vi "Find Analog Replay.vi"(8 "error in (no error)":errorcluster, 9 "RIO Device Address":string, 10 "Name":string, 11 "APU in":refnum<k24>) -> (0 "error out":errorcluster, 2 "Analog Replay":refnum<k24>, 3 "APU out":refnum<k24>)   [LabVIEW 2020, in "Engine Simulation Toolkit Scripting API.lvlib"]
uses:
  Engine Simulation Toolkit Scripting API.lvlib
  NationalInstruments.VeriStand.SystemDefinitionAPI
  Shared/Constants and GUIDs.vi
  Shared/Engine Simulation Toolkit Shared.lvlib
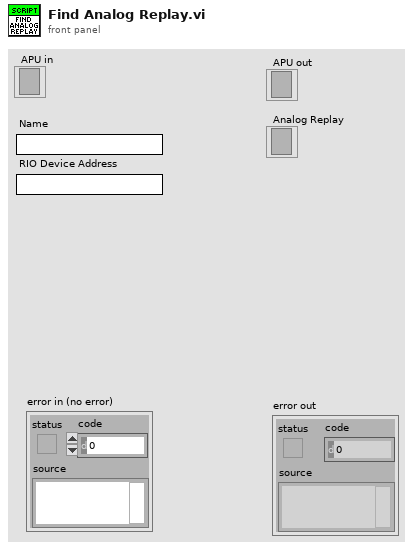
[diagram p1: front panel]
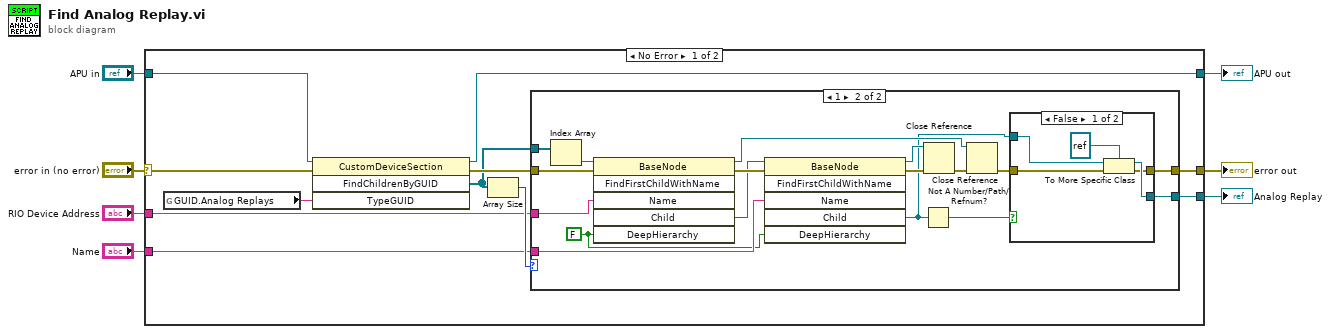
[diagram p0: block diagram]
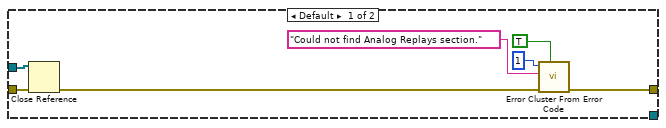
[diagram p2: hidden frame]
diagram:
  n1 = case shown="No Error" "error in (no error)" {
    selector: "error in (no error)" -> [w10 w50]
    tunnel: [w12 w50] -> w7
    tunnel: "APU in" -> [w18 w49]
    tunnel: [w11 w49] -> w4
    tunnel: "RIO Device Address" -> [w13 _]
    tunnel: "Name" -> [w9 _]
    tunnel: [w8 _] -> w1
    frame No Error {
      n2 = global read "Constants and GUIDs.vi" "GUID.Analog Replays"() -> (w17:string)
      n3 = invoke class="CustomDeviceSection" method="FindChildrenByGUID"(reference=w18, error in=w10, "TypeGUID"=w17) -> (reference out=w11:refnum<k24>, error out=w15:errorcluster, "FindChildrenByGUID"=w14:refnum<k24>[])  [unwired: 1 in, 1 out]
      n4 = Array Size(array=w14) -> (size(s)=w16:i32)
      n5 = case shown="1" w16 {
        tunnel: [w25 w27] -> w12
        tunnel: w15 -> [w20 w37]
        tunnel: w14 -> [w21 w42]
        tunnel: w13 -> [_ w40]
        tunnel: w9 -> [_ w32]
        tunnel: [_ w26] -> w8
        frame Default {
          n6 = Close Reference(reference=w21, error in (no error)=w20) -> (error out=w19:errorcluster)
          n7 = call <vilib>:"Error Cluster From Error Code.vi"("show call chain? (False)"=TRUE, "error in (no error)"=w19, "error message (\"\")"="Could not find Analog Replays section." ("error message (\"\")"), "error code (0)"=1) -> ("error out"=w25:errorcluster)  [unwired: 5 in]
        }
        frame 1 {
          w31 = FALSE ("DeepHierarchy")
          n8 = Index Array(array=w42) -> (element=w41:refnum<k24>)  [unwired: 1 in]
          n9 = invoke class="BaseNode" method="FindFirstChildWithName"(reference=w41, error in=w37, "Name"=w40, "DeepHierarchy"=w31) -> (reference out=w33:refnum<k24>, error out=w39:errorcluster, "Child"=w38:refnum<k24>)  [unwired: 2 in, 3 out]
          n10 = invoke class="BaseNode" method="FindFirstChildWithName"(reference=w38, error in=w39, "Name"=w32, "DeepHierarchy"=w31) -> (reference out=w36:refnum<k24>, error out=w35:errorcluster, "Child"=w29:refnum<k24>)  [unwired: 2 in, 3 out]
          n11 = Not A Number/Path/Refnum?(number/path/refnum=w29) -> (NaN/Path/Refnum?=w30:bool)
          n12 = Close Reference(reference=w36, error in (no error)=w35) -> (error out=w34:errorcluster)
          n13 = Close Reference(reference=w33, error in (no error)=w34) -> (error out=w28:errorcluster)
          n14 = case shown="False" w30 {
            tunnel: [w47 _] -> w26
            tunnel: w28 -> [w46 w48]
            tunnel: [w45 w48] -> w27
            tunnel: w29 -> [w43 _]
            frame False {
              n15 = To More Specific Class(target class=refnum<k24> refnum ("APU"), reference=w43, error in=w46) -> (specific class reference=w47:refnum<k24>, error out=w45:errorcluster)
            }
            frame True {
            }
          }
        }
      }
    }
    frame Error {
    }
  }
  "error out" <- w7
  "APU out" <- w4
  "Analog Replay" <- w1
